vi "strings to line.vi"(11 "strings":string[](array[string])) -> (3 "line":T3)   [LabVIEW 2015, in "Modbus Module editor node.lvclass"]
doc: "Platypus Framework 1.0.1.65\nNI Systems Engineering - National Instruments"
uses:
  Modbus Module editor node.lvclass
  table line.ctl
  module/module channel/Modbus Module Channel.lvclass
  <vilib>/NI/Tag Bus Module Framework/channel/channel classification.ctl
  permissions.ctl
  <vilib>/NI/Tag Bus/tag/Data Type.ctl
  <vilib>/NI/Tag Bus/tag/tag descriptor.lvclass/tag descriptor.ctl
  <vilib>/NI/Tag Bus Module Framework/channel/TBM channel.lvclass/TBM channel.ctl
  <vilib>/NI/Tag Bus/tag/write tag name.vi
  <vilib>/NI/Tag Bus Module Framework/channel/Write channel classification.vi
  <vilib>/NI/Tag Bus/tag/write data type.vi
  <vilib>/NI/Tag Bus/tag/tag descriptor.lvclass
  <vilib>/NI/Tag Bus Module Framework/channel/TBM channel.lvclass
panel:
  in  "display permissions":T1
  in  "channel classification":T2
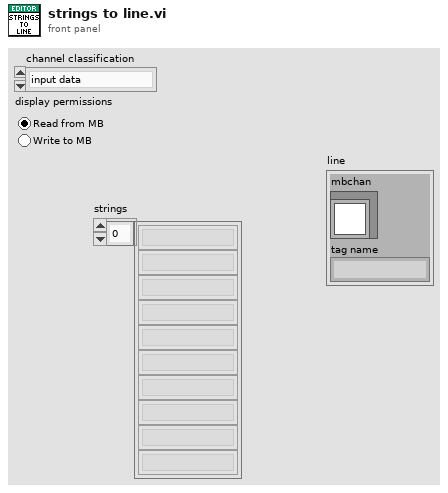
[diagram p1: front panel]
types:
  T1 = typedef "Modbus Module editor node.lvclass/permissions.ctl" = enum32{"Read from MB", "Write to MB"}
  T2 = typedef "TBM channel.lvclass/channel classification.ctl" = enum16{"input data", "output data", "processing parameter", "processing result"}
  T3 = typedef "Modbus Module editor node.lvclass/table line.ctl" = cluster{"mbchan":refnum<class "Modbus Module Channel.lvclass">, "tag name":string}
  T4 = typedef "tag bus.lvlib/tag descriptor.lvclass/Data Type.ctl" = enum16{"Double", "Single", "I64", "I32", "I16", "I8", "U64", "U32", "U16", "U8", "Boolean", "String", "Array of Double", "Array of Single", "Array of I64", "Array of I32", "Array of I16", "Array of I8", "Array of U64", "Array of U32", "Array of U16", "Array of U8", "Array of Boolean", "Array of String"}
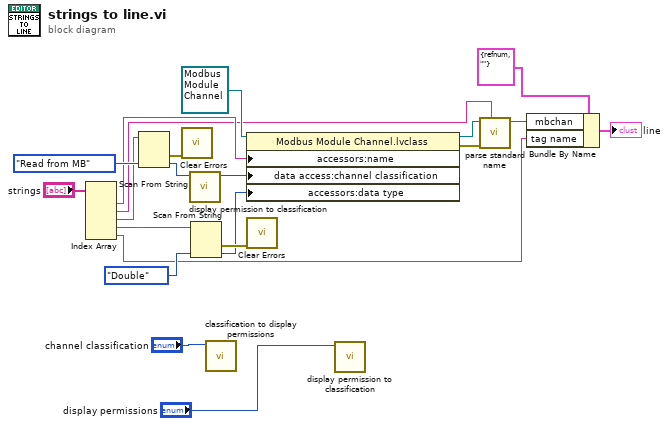
[diagram p0: block diagram]
diagram:
  n1 = Index Array(array="strings") -> (element #1=w10:string, element #2=w6:string, element #3=w5:string, element #4=w4:string, element #5=w3:string)  [unwired: 5 in]
  n2 = Scan From String(input string=w5, default 1=permissions."Read from MB" ("direction")) -> (error out=w16:errorcluster, output 1=w14:T1)  [unwired: 3 in, 2 out]
  n3 = call <vilib>:"Clear Errors.vi"("error in (no error)"=w16) -> ()  [unwired: 5 in, 2 out]
  n4 = call "display permission to classification.vi"("display permissions"=w14) -> ("channel classification"=w11:T2)  [unwired: 10 in]
  n5 = Scan From String(input string=w4, default 1=Data_Type."Double" ("data type")) -> (error out=w18:errorcluster, output 1=w12:T4)  [unwired: 3 in, 2 out]
  n6 = call "classification to display permissions.vi"("channel classification"="channel classification") -> ()  [unwired: 10 in, 1 out]
  n7 = property class="Modbus Module Channel.lvclass"(reference=refnum<class "Modbus Module Channel.lvclass"> refnum ("Modbus Module Channel"), "accessors:name"=w10, "data access:channel classification"=w11, "accessors:data type"=w12) -> (reference out=w9:refnum<class "Modbus Module Channel.lvclass">, error out=w8:errorcluster)  [unwired: 1 in]
  n8 = call <vilib>:"Clear Errors.vi"("error in (no error)"=w18) -> ()  [unwired: 5 in, 2 out]
  n9 = call "display permission to classification.vi"("display permissions"="display permissions") -> ()  [unwired: 10 in, 1 out]
  n10 = call "parse standard name.vi"("standard name"=w6, "error in"=w8, "Modbus Module Channel in"=w9) -> ("Modbus Module Channel out"=w7:refnum<class "Modbus Module Channel.lvclass">)  [unwired: 7 in, 1 out]
  n11 = Bundle By Name(cluster=T3 {"mbchan"=refnum, "tag name"=""} ("line"), "mbchan"=w7, "tag name"=w3) -> (→"line":T3)
